vi "CE Examples Navigator.vi"() -> ()   [LabVIEW 2021]
doc: "::: CalcExpress Toolkit :::\nCopyright (c) 2000-2026 Konstantin Shifershteyn. All rights reserved."
uses:
  vi.lib/addons/CalcExpress/cemisc.llb/[ce] CE component paths - Kind of Path Enum.ctl
panel:
  in  "Tree":string(tree) caption="Double-click an example to open"
  in  "Note":string="1)  Interactive Script Processor (CSE ISP) also contains examples. Run it and select Examples menu.\n2)  Many examples use Advanced Analysis VIs. These examples don't work properly if you don't have these VIs."
  out "Description":string
  in  "Mass Compile":bool
  in  "Run CSE ISP":bool
  in  "EXIT":bool
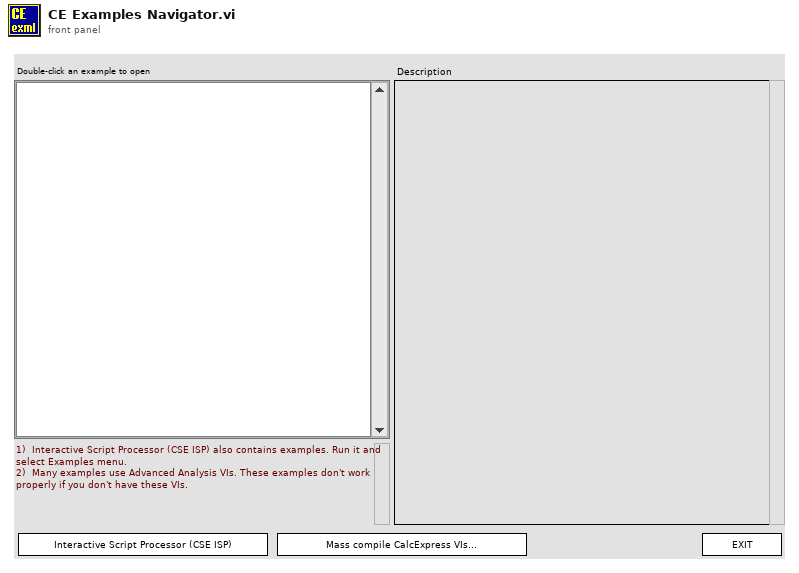
[diagram p1: front panel]
types:
  T1 = typedef "[ce] CE component paths - Kind of Path Enum.ctl" = enum16{"VIs", "FuncVIs", "Help", "Examples", "Project", "Templates"}
  T2 = enum32{"invalid app kind", "Development System", "Run Time System", "Student Edition", "Embedded LabVIEW", "Evaluation", "Custom"}
  T3 = typedef "eventvkey.ctl" = enum16{"ASCII", "Enter", "Return", "Shift", "Ctrl", "Alt", "Cmd", "Opt", "Caps", "NumLock", "Clear", "Break", "Up", "Down", "Left", "Right", "Insert", "Delete", "Home", "End", "PageUp", "PageDown", "Escape", "Help", "Pause", "ScrollLock", "F1", "F2", "F3", "F4", "F5", "F6", "F7", "F8", "F9", "F10", "F11", "F12", "F13", "F14", "F15", "F16", "F17", "F18", "F19", "F20", "F21", "F22", "F23", "F24", "Play", "VolumeUp", "VolumeDown", "Mute", "Two Byte Char"}
  T4 = cluster{"Shift":bool, "Ctrl":bool, "Alt":bool, "Cmd":bool, "Opt":bool}
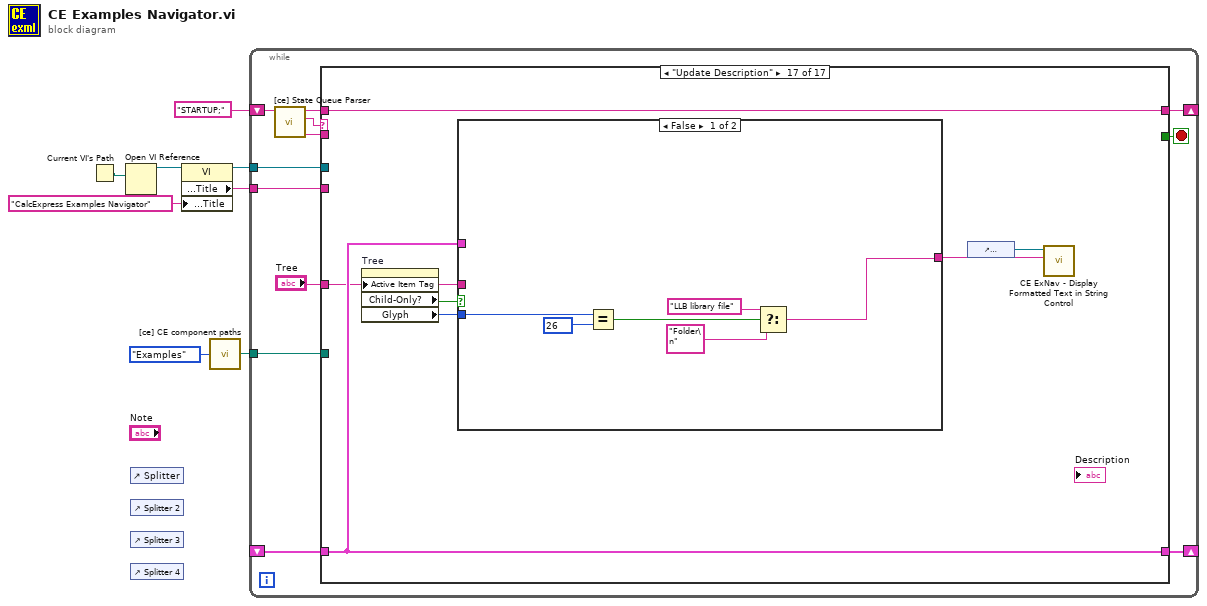
[diagram p0: block diagram]
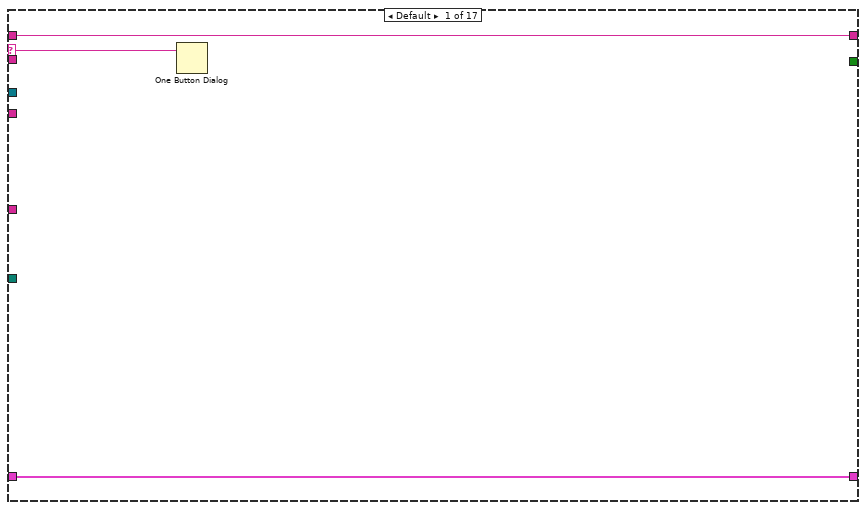
[diagram p2: hidden frame]
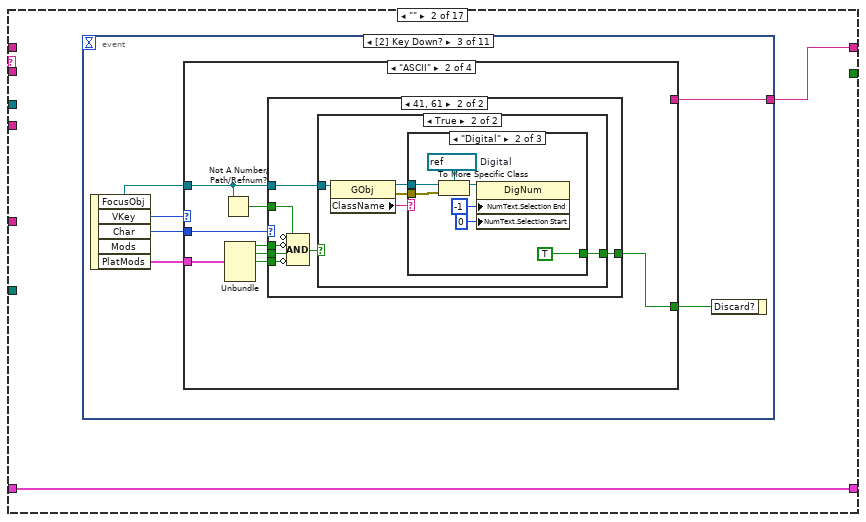
[diagram p3: hidden frame]
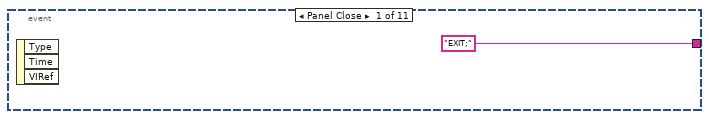
[diagram p4: hidden frame]
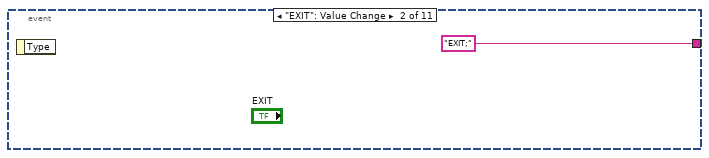
[diagram p5: hidden frame]
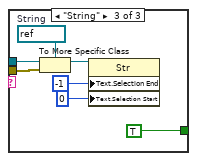
[diagram p10: hidden frame]
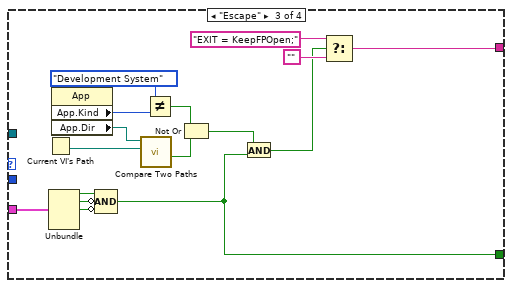
[diagram p11: hidden frame]
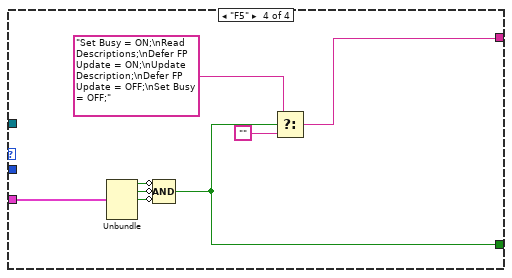
[diagram p12: hidden frame]
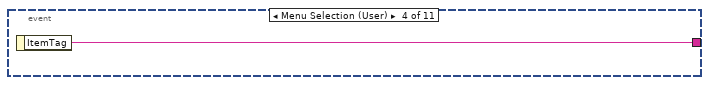
[diagram p13: hidden frame]
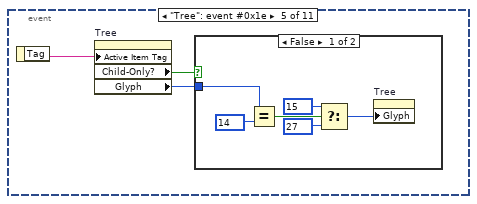
[diagram p14: hidden frame]
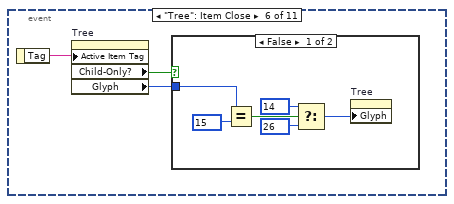
[diagram p16: hidden frame]
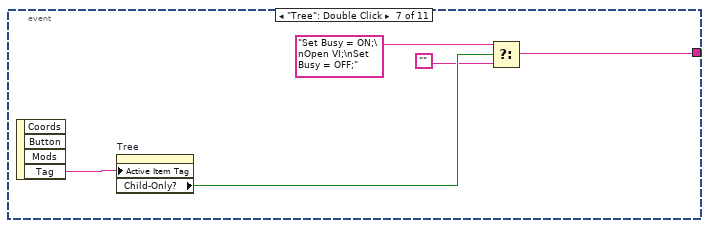
[diagram p18: hidden frame]
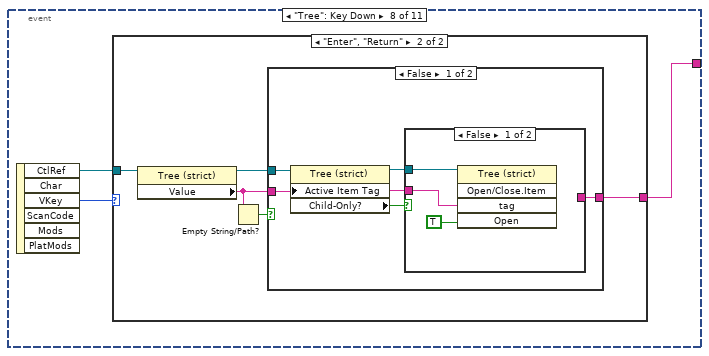
[diagram p19: hidden frame]
diagram:
  n1 = Current VI's Path() -> (path=w6:path)
  n2 = Open VI Reference(vi path=w6) -> (vi reference=w5:refnum<vi>)  [unwired: 5 in, 1 out]
  n3 = control-ref of="Splitter"() -> ()  [unwired: 1 out]
  n4 = control-ref of="Splitter 2"() -> ()  [unwired: 1 out]
  n5 = control-ref of="Splitter 3"() -> ()  [unwired: 1 out]
  n6 = control-ref of="Splitter 4"() -> ()  [unwired: 1 out]
  n7 = property class="VI"(reference=w5, "Front Panel.Title"="CalcExpress Examples Navigator" ("Front Panel Window:Title")) -> (reference out=w4:refnum<vi>, "Front Panel.Title"=w3:string)  [unwired: 1 in, 1 out]
  n8 = call "[ce] CE component paths.vi"("kind of path"=[ce]_CE_component_paths_-_Kind_of_Path_Enum."Examples") -> ("path out"=w7:path)  [unwired: 1 in]
  n9 = while {
    shift-right: [w18] -> _
    shift-left: "STARTUP;" -> [w20]
    tunnel: w7 -> [w14]
    shift-right: [w13] -> _
    shift-left: _ -> [w12]
    tunnel: w4 -> [w10]
    tunnel: w3 -> [w9]
    stop <- w16 stop-if-true
    n10 = call "[ce] State Queue Parser.vi"("input queue"=w20) -> ("state parameters"=w15:string, "state"=w19:string, "remained queue"=w17:string)  [unwired: 6 in]
    n11 = case shown="\"Update Description\"" w19 {
      selector: w19 -> [w22 _ _ _ _ _ _ _ _ _ _ _ _ _ _ _ _]
      tunnel: [w23 w25 "Set Busy = ON;\n\nINIT;\n\nSet Busy = OFF;" w150 w158 w171 w175 w181 w185 w190 w193 w214 w217 w251 w265 w271 w283] -> w18
      tunnel: w17 -> [w23 _ _ w151 w158 w171 w175 w181 w185 w190 w193 w214 w224 w251 w265 w271 w283]
      tunnel: [_ _ _ _ _ TRUE _ _ _ _ _ _ _ _ _ _ _] -> w16
      tunnel: w15 -> [_ _ _ _ _ w169 _ w179 w184 _ w191 _ _ _ _ _ _]
      tunnel: w14 -> [_ _ _ w143 _ _ _ _ _ _ _ _ w223 _ _ _ _]
      tunnel: [w21 w24 w137 w142 w159 w168 w176 w177 w183 w189 w192 w215 w222 w250 w266 w267 w282] -> w13
      tunnel: w12 -> [w21 w24 w137 _ w159 w168 w176 w177 w183 w189 w192 w215 w222 w250 w266 w269 w282]
      tunnel: "Tree" -> [_ _ _ _ _ _ _ _ _ w188 _ _ _ _ _ _ w279]
      tunnel: w10 -> [_ _ _ _ _ w162 _ _ _ _ _ _ _ _ _ _ _]
      tunnel: w9 -> [_ _ _ _ _ w160 _ _ _ _ _ _ _ _ _ _ _]
      frame Default {
        n12 = One Button Dialog(message=w22) -> ()  [unwired: 1 in, 1 out]
      }
      frame "" {
        n13 = event shown="[2] Key Down?" {
          selector: _ -> [_ _ _ _ _ _ _ _ _ _ _]
          dyn-events: _ -> [_ _ _ _ _ _ _ _ _ _ _]
          timeout: _ -> [_ _ _ _ _ _ _ _ _ _ _]
          tunnel: ["EXIT;" "EXIT;" w32 w92 _ _ w113 w116 "Defer FP Update = ON;\nUpdate Description;\nDefer FP Update = OFF;" "Menu = CSE ISP;" ("ItemTag") "Menu = Mass Compile;" ("ItemTag")] -> w25
          event Panel Close {
            n14 = event-data() -> ()  [unwired: 1 in, 3 out]
          }
          event "EXIT": Value Change {
            n15 = event-data() -> ()  [unwired: 1 in, 1 out]
          }
          event Key Down? {
            n16 = event-data() -> ("FocusObj"=w28:refnum<vi>, "VKey"=w30:T3, "Char"=w29:i16, "PlatMods"=w33:T4)  [unwired: 1 in, 1 out]
            n17 = case shown="\"ASCII\"" w30 {
              tunnel: w33 -> [_ w37 w78 w86]
              tunnel: [_ _ w77 w85] -> w32
              tunnel: [_ w35 w69 w84] -> w31
              tunnel: w29 -> [_ w36 _ _]
              tunnel: w28 -> [_ w34 _ _]
              frame Default {
              }
              frame "ASCII" {
                n18 = Not A Number/Path/Refnum?(number/path/refnum=w34) -> (NaN/Path/Refnum?=w41:bool)
                n19 = Unbundle(w37) -> ("Shift"=w38:bool, "Ctrl"=w39:bool, "Alt"=w40:bool)  [unwired: 2 out]
                n20 = case shown="41, 61" w36 {
                  tunnel: w38 -> [_ w48]
                  tunnel: w39 -> [_ w47]
                  tunnel: w40 -> [_ w46]
                  tunnel: w34 -> [_ w44]
                  tunnel: [_ w43] -> w35
                  tunnel: w41 -> [_ w42]
                  frame Default {
                  }
                  frame 65, 97 {
                    n21 = Compound Arithmetic op=AND(invert w42, invert w48, w47, invert w46) -> (w45:bool)
                    n22 = case shown="True" w45 {
                      tunnel: w44 -> [_ w53]
                      tunnel: [_ w51] -> w43
                      frame False {
                      }
                      frame True {
                        n23 = property class="GObj"(reference=w53) -> (reference out=w50:refnum<vi>, error out=w49:errorcluster, "ClassName"=w52:string)  [unwired: 1 in]
                        n24 = case shown="\"Digital\"" w52 {
                          tunnel: [_ TRUE TRUE] -> w51
                          tunnel: w50 -> [_ w58 w65]
                          tunnel: w49 -> [_ w57 w64]
                          frame Default {
                          }
                          frame "Digital" {
                            w59 = refnum<vi> refnum  # Digital
                            n25 = To More Specific Class(target class=w59, reference=w58, error in=w57) -> (specific class reference=w56:refnum<vi>)  [unwired: 1 out]
                            n26 = property class="DigNum"(reference=w56, "NumText.Selection End"=-1 ("Numeric Text.Selection:End"), "NumText.Selection Start"=u32 0 ("Numeric Text.Selection:Start")) -> ()  [unwired: 1 in, 2 out]
                          }
                          frame "String" {
                            w66 = refnum<vi> refnum  # String
                            n27 = To More Specific Class(target class=w66, reference=w65, error in=w64) -> (specific class reference=w63:refnum<vi>)  [unwired: 1 out]
                            n28 = property class="Str"(reference=w63, "Text.Selection End"=-1 ("Numeric Text.Selection:End"), "Text.Selection Start"=u32 0 ("Numeric Text.Selection:Start")) -> ()  [unwired: 1 in, 2 out]
                          }
                        }
                      }
                    }
                  }
                }
              }
              frame "Escape" {
                n29 = Current VI's Path() -> (path=w76:path)
                n30 = Unbundle(w78) -> ("Shift"=w79:bool, "Ctrl"=w80:bool, "Alt"=w81:bool)  [unwired: 2 out]
                n31 = property class="App"() -> ("App.Kind"=w74:T2, "App.Dir"=w75:path)  [unwired: 2 in, 2 out]
                n32 = Compound Arithmetic op=AND(w79, invert w80, invert w81) -> (w69:bool)
                n33 = call <vilib>:"Compare Two Paths.vi"("Path 2"=w76, "Path 1"=w75) -> ("Path 2 Relative to Path 1?"=w72:bool)  [unwired: 6 in, 3 out]
                n34 = Not Equal?(x=T2."Development System", y=w74) -> (x != y?=w73:bool)
                n35 = Not Or(1:w72, 2:w73) -> (0:w71:bool)
                n36 = And(x=w71, y=w69) -> (x .and. y?=w68:bool)
                n37 = Select(t="EXIT = KeepFPOpen;", s=w68, f="") -> (s? t:f=w77:string)
              }
              frame "F5" {
                n38 = Unbundle(w86) -> ("Shift"=w87:bool, "Ctrl"=w88:bool, "Alt"=w89:bool)  [unwired: 2 out]
                n39 = Compound Arithmetic op=AND(invert w87, invert w88, invert w89) -> (w84:bool)
                n40 = Select(t="Set Busy = ON;\nRead Descriptions;\nDefer FP Update = ON;\nUpdate Description;\nDefer FP Update = OFF;\nSet Busy = OFF;", s=w84, f="") -> (s? t:f=w85:string)
              }
            }
            n41 = event-data("Discard?"=w31) -> ()  [unwired: 1 in, 1 out]
          }
          event Menu Selection (User) {
            n42 = event-data() -> ("ItemTag"=w92:string)  [unwired: 1 in]
          }
          event "Tree": event #0x1e {
            n43 = event-data() -> ("Tag"=w95:string)  [unwired: 1 in]
            n44 = property on="Tree" class="Tree (strict)"("Active Item Tag"=w95) -> ("Child-Only?"=w93:bool, "Glyph"=w94:i32)  [unwired: 2 in, 2 out]
            n45 = case shown="False" w93 {
              tunnel: w94 -> [w101 _]
              frame False {
                n46 = Equal?(x=w101, y=14) -> (x = y?=w99:bool)
                n47 = Select(t=15, s=w99, f=27) -> (s? t:f=w98:i32)
                n48 = property on="Tree" class="Tree (strict)"("Glyph"=w98) -> ()  [unwired: 2 in, 2 out]
              }
              frame True {
              }
            }
          }
          event "Tree": Item Close {
            n49 = event-data() -> ("Tag"=w102:string)  [unwired: 1 in]
            n50 = property on="Tree" class="Tree (strict)"("Active Item Tag"=w102) -> ("Child-Only?"=w103:bool, "Glyph"=w104:i32)  [unwired: 2 in, 2 out]
            n51 = case shown="False" w103 {
              tunnel: w104 -> [w110 _]
              frame False {
                n52 = Equal?(x=w110, y=15) -> (x = y?=w108:bool)
                n53 = Select(t=14, s=w108, f=26) -> (s? t:f=w107:i32)
                n54 = property on="Tree" class="Tree (strict)"("Glyph"=w107) -> ()  [unwired: 2 in, 2 out]
              }
              frame True {
              }
            }
          }
          event "Tree": Double Click {
            n55 = event-data() -> ("Tag"=w115:string)  [unwired: 1 in, 3 out]
            n56 = property on="Tree" class="Tree (strict)"("Active Item Tag"=w115) -> ("Child-Only?"=w114:bool)  [unwired: 2 in, 2 out]
            n57 = Select(t="Set Busy = ON;\nOpen VI;\nSet Busy = OFF;", s=w114, f="") -> (s? t:f=w113:string)
          }
          event "Tree": Key Down {
            n58 = event-data() -> ("CtlRef"=w118:refnum<vi>, "VKey"=w117:T3)  [unwired: 1 in, 4 out]
            n59 = case shown="\"Enter\", \"Return\"" w117 {
              tunnel: w118 -> [_ w123]
              tunnel: [_ w119] -> w116
              frame Default {
              }
              frame "Enter", "Return" {
                n60 = property class="Tree (strict)"(reference=w123) -> (reference out=w122:refnum<vi>, "Value"=w120:string)  [unwired: 1 in, 1 out]
                n61 = Empty String/Path?(string/path=w120) -> (empty?=w121:bool)
                n62 = case shown="False" w121 {
                  tunnel: w122 -> [w128 _]
                  tunnel: w120 -> [w124 _]
                  tunnel: [w125 _] -> w119
                  frame False {
                    n63 = property on="Property Node" class="Tree (strict)"(reference=w128, "Active Item Tag"=w124) -> (reference out=w127:refnum<vi>, "Child-Only?"=w126:bool)  [unwired: 1 in, 1 out]
                    n64 = case shown="False" w126 {
                      tunnel: w127 -> [w131 _]
                      tunnel: [_ "Set Busy = ON;\nOpen VI;\nSet Busy = OFF;"] -> w125
                      tunnel: w124 -> [w129 _]
                      frame False {
                        n65 = invoke class="Tree (strict)" method="Open/Close.Item"(reference=w131, "tag"=w129, "Open"=TRUE) -> ()  [unwired: 2 in, 5 out]
                      }
                      frame True {
                      }
                    }
                  }
                  frame True {
                  }
                }
              }
            }
          }
          event "Tree": Value Change {
            (unwired) "Set Busy = ON;\nUpdate Description;\nSet Busy = OFF;"
            n66 = event-data() -> ()  [unwired: 1 in, 2 out]
          }
          event "Run CSE ISP": Value Change {
            n67 = event-data() -> ()  [unwired: 1 in, 1 out]
          }
          event "Mass Compile": Value Change {
            n68 = event-data() -> ()  [unwired: 1 in, 1 out]
          }
        }
      }
      frame "STARTUP" {
      }
      frame "INIT" {
        n69 = Build Array("[ex ce*.vi" ("pattern"), "FuncVI-*.vi" ("pattern")) -> (w146:string[])
        n70 = for {
          tunnel: w143 -> [w157]
          tunnel: w146 -> [w155] mode=indexing
          shift-right: [w152] -> w148
          shift-left: path[] [] -> [w153]
          n71 = call <vilib>:"Recursive File List.vi"("pattern"=w155, "Treat LLBs as Folders?"=TRUE, "Folder Path"=w157) -> ("All Files in Dir"=w154:path[])  [unwired: 4 in, 4 out]
          n72 = Build Array (concatenate)(w153, w154) -> (w152:path[])
        }
        n73 = Sort 1D Array(array=w148) -> (sorted array=w139:path[])
        n74 = Array Size(array=w139) -> (size(s)=w140:i32)
        n75 = Initialize Array("", w140) -> (w138:string[])
        n76 = Bundle(w139, w138) -> (w142:cluster{path[], string[]})  [unwired: 1 in]
        n77 = Concatenate Strings("Defer FP Update = ON;\nRead Descriptions;\nBuild Tree;\nDefer FP Update = OFF;\n\nInit Done;", w151) -> (w150:string)
      }
      frame "INIT Done" {
      }
      frame "EXIT" {
        n78 = property class="VI"(reference=w162, "Front Panel.Title"=w160) -> (reference out=w161:refnum<vi>)  [unwired: 1 in, 1 out]
        n79 = case shown="Default" w169 {
          tunnel: w161 -> [w172 w174]
          tunnel: [w172 w173] -> w164
          frame "KeepFPOpen" {
          }
          frame Default {
            n80 = invoke class="VI" method="FP.Close"(reference=w174) -> (reference out=w173:refnum<vi>)  [unwired: 2 in, 2 out]
          }
        }
        n81 = local write "Description"("") -> ()
        n82 = invoke on="Tree" class="Tree (strict)" method="Edit Tree Items.Delete"("tag"="", "Delete Children"=TRUE ("Delete Children?")) -> (error out=w163:errorcluster)  [unwired: 3 in, 4 out]
        n83 = Close Reference(reference=w164, error in (no error)=w163) -> ()  [unwired: 1 out]
      }
      frame "---------------------------------- 1" {
      }
      frame "Defer FP Update" {
        n84 = case shown="\"ON\"" w179 {
          tunnel: [_ TRUE] -> w178
          frame "OFF", Default {
          }
          frame "ON" {
          }
        }
        n85 = property class="VI"() -> ("Front Panel"=w180:refnum<vi>)  [unwired: 2 in, 2 out]
        n86 = property class="Pnl"(reference=w180, "Defer Panel Updates"=w178) -> ()  [unwired: 1 in, 2 out]
      }
      frame "Set Busy" {
        n87 = case shown="\"ON\"" w184 {
          frame "OFF", Default {
            n88 = call <vilib>:"Unset Busy.vi"() -> ()  [unwired: 11 in, 1 out]
          }
          frame "ON" {
            n89 = call <vilib>:"Set Busy.vi"() -> ()  [unwired: 10 in, 2 out]
          }
        }
      }
      frame "Open VI" {
        n90 = String To Path(string=w188) -> (path=w186:path)
        n91 = call "CE ExNav - VIs Control.vi"("cmd"=enum16{"open", "run", "description"}."open", "VI path"=w186) -> ()  [unwired: 8 in, 2 out]
      }
      frame "Menu" {
        n92 = case shown="\"About\"" w191 {
          frame Default {
          }
          frame "About" {
            n93 = call "[ce] MsgBox - About CalcExpress.vi"() -> ()  [unwired: 11 in, 1 out]
          }
          frame "CE Help" {
            n94 = call "[ce] CE component paths.vi"("kind of path"=[ce]_CE_component_paths_-_Kind_of_Path_Enum."Help", "append path"="CEToolkit.chm" ("append")) -> ("path out"=w196:path)
            n95 = Control Online Help(2:w196, 4:enum16{"Contents", "Key", "Close"}."Contents" ("Operation")) -> (0:w197:errorcluster)  [unwired: 2 in]
            n96 = call <vilib>:"Simple Error Handler.vi"("error in (no error)"=w197) -> ()  [unwired: 4 in, 5 out]
          }
          frame "CSE ISP" {
            n97 = call "[ce] CE component paths.vi"("kind of path"=[ce]_CE_component_paths_-_Kind_of_Path_Enum."Project", "append path"="CSE ISP.vi" ("append")) -> ("path out"=w200:path)
            n98 = call "CE ExNav - VIs Control.vi"("cmd"=enum16{"open", "run", "description"}."run", "VI path"=w200) -> ("error out"=w202:errorcluster)  [unwired: 8 in, 1 out]
            n99 = call <vilib>:"Simple Error Handler.vi"("error in (no error)"=w202) -> ()  [unwired: 4 in, 5 out]
          }
          frame "VarMan Spy" {
            n100 = call "[ce] CE component paths.vi"("kind of path"=[ce]_CE_component_paths_-_Kind_of_Path_Enum."Project", "append path"="VarMan Spy.vi" ("append")) -> ("path out"=w208:path)
            n101 = call "CE ExNav - VIs Control.vi"("cmd"=enum16{"open", "run", "description"}."run", "VI path"=w208) -> ("error out"=w206:errorcluster)  [unwired: 8 in, 1 out]
            n102 = call <vilib>:"Simple Error Handler.vi"("error in (no error)"=w206) -> ()  [unwired: 4 in, 5 out]
          }
          frame "Mass Compile" {
            n103 = call "[ce] CE component paths.vi"("kind of path"=[ce]_CE_component_paths_-_Kind_of_Path_Enum."Project", "append path"="Mass Compile CalcExpress VIs.vi" ("append")) -> ("path out"=w213:path)
            n104 = call "CE ExNav - VIs Control.vi"("cmd"=enum16{"open", "run", "description"}."run", "VI path"=w213) -> ("error out"=w211:errorcluster)  [unwired: 8 in, 1 out]
            n105 = call <vilib>:"Simple Error Handler.vi"("error in (no error)"=w211) -> ()  [unwired: 4 in, 5 out]
          }
        }
      }
      frame "---------------------------------- 2" {
      }
      frame "Build Tree" {
        n106 = Unbundle(w222) -> (w221:path[])  [unwired: 1 out]
        n107 = invoke on="Tree" class="Tree (strict)" method="Edit Tree Items.Delete"("tag"="", "Delete Children"=TRUE ("Delete Children?")) -> (error out=w218:errorcluster)  [unwired: 3 in, 4 out]
        n108 = for {
          tunnel: w221 -> [w229] mode=indexing
          tunnel: w223 -> [w226]
          tunnel: w218 -> [_]
          n109 = Path To String(path=w226) -> (string=w225:string)
          n110 = call <vilib>:"Compare Two Paths.vi"("Path 2"=w229, "Path 1"=w226) -> ("Relative Path from 1 to 2"=w228:path)  [unwired: 6 in, 3 out]
          n111 = Path to Array of Strings(0:w228) -> (2:w227:string[])  [unwired: 1 out]
          n112 = for {
            N -> [w232]
            tunnel: w227 -> [w240] mode=indexing
            shift-right: [w241] -> _
            shift-left: w225 -> [w237]
            i -> [w233]
            n113 = Decrement(x=w232) -> (x-1=w231:i32)
            n114 = Concatenate Strings(w237, "\\" ("string"), w240) -> (w235:string)
            n115 = Equal?(x=w231, y=w233) -> (x = y?=w230:bool)
            n116 = Equal To 0?(x=w233) -> (x = 0?=w238:bool)
            n117 = property on="Tree" class="Tree (strict)"("Active Item Tag"=w235) -> (error out=w234:errorcluster)  [unwired: 2 in, 1 out]
            n118 = Select(t="", s=w238, f=w237) -> (s? t:f=w239:string)
            n119 = case shown="No Error" w234 {
              tunnel: [w243 w249] -> w241
              tunnel: w240 -> [_ w248]
              tunnel: w239 -> [_ w246]
              tunnel: w235 -> [w243 w245]
              tunnel: w230 -> [_ w244]
              frame No Error {
              }
              frame Error {
                n120 = invoke on="Tree" class="Tree (strict)" method="Edit Tree Items.Add Item"("Parent Tag"=w246, "Child Position"=-1, "Left Cell"=w248, "Child Tag"=w245, "Child Only?"=w244) -> ("Edit Tree Items:Add Item"=w249:string)  [unwired: 4 in, 8 out]
              }
            }
          }
        }
        n121 = Concatenate Strings("Build Tree 2;" ("string"), w224) -> (w217:string)
      }
      frame "Build Tree 2" {
        n122 = invoke on="Tree" class="Tree (strict)" method="Open/Close.Open/Close All"("Open"=FALSE ("Open?")) -> (error out=w252:errorcluster)  [unwired: 3 in, 3 out]
        n123 = property on="Tree" class="Tree (strict)"(error in=w252) -> ("All Tags"=w254:string[])  [unwired: 1 in, 2 out]
        n124 = for {
          tunnel: w254 -> [w259] mode=indexing
          n125 = String To Path(string=w259) -> (path=w260:path)
          n126 = property on="Tree" class="Tree (strict)"("Active Item Tag"=w259) -> (error out=w262:errorcluster, "Child-Only?"=w264:bool)  [unwired: 2 in, 1 out]
          n127 = File/Directory Info(path=w260) -> (directory=w258:bool)  [unwired: 1 in, 6 out]
          n128 = Select(t=14, s=w258, f=26) -> (s? t:f=w257:i32)
          n129 = Select(t=21, s=w264, f=w257) -> (s? t:f=w261:i32)
          n130 = property on="Tree" class="Tree (strict)"(error in=w262, "Glyph"=w261) -> ()  [unwired: 1 in, 2 out]
        }
      }
      frame "---------------------------------- 3" {
      }
      frame "Read Descriptions" {
        n131 = Unbundle(w269) -> (w270:path[])  [unwired: 1 out]
        n132 = for {
          tunnel: w270 -> [w275] mode=indexing
          tunnel: [w273] -> w268 mode=indexing
          n133 = call "CE ExNav - VIs Control.vi"("cmd"=enum16{"open", "run", "description"}."description", "VI path"=w275) -> ("description"=w274:string)  [unwired: 8 in, 1 out]
          n134 = Match Pattern(string=w274, regular expression="\\n:::") -> (before substring=w273:string)  [unwired: 1 in, 3 out]
        }
        n135 = Bundle(cluster=w269, w268) -> (w267:cluster{path[], string[]})  [unwired: 1 in]
      }
      frame "Update Description" {
        n136 = property on="Tree" class="Tree (strict)"("Active Item Tag"=w279) -> ("Child-Only?"=w278:bool, "Glyph"=w277:i32)  [unwired: 2 in, 2 out]
        n137 = case shown="False" w278 {
          tunnel: w282 -> [_ w306]
          tunnel: [w287 w291] -> w280
          tunnel: w279 -> [_ w290]
          tunnel: w277 -> [w286 _]
          frame False {
            n138 = Equal?(x=w286, y=26) -> (x = y?=w284:bool)
            n139 = Select(t="LLB library file", s=w284, f="Folder\n") -> (s? t:f=w287:string)
          }
          frame True {
            n140 = Unbundle(w306) -> (w305:path[], w303:string[])
            n141 = String To Path(string=w290) -> (path=w296:path)
            n142 = Search 1D Array(1D array=w305, element=w296) -> (index of element=w304:i32)  [unwired: 1 in]
            n143 = Index Array(array=w303, index=w304) -> (element=w297:string)
            n144 = Strip Path(path=w296) -> (name=w295:string)  [unwired: 1 out]
            n145 = Empty String/Path?(string/path=w297) -> (empty?=w302:bool)
            n146 = Not(x=w302) -> (.not. x?=w301:bool)
            n147 = Format Into String(format string="<B>%s</B>\n\n", w295) -> (resulting string=w293:string)  [unwired: 2 in, 1 out]
            n148 = Match Pattern(string=w297, regular expression="^<[Bb]>") -> (offset past match=w298:i32)  [unwired: 1 in, 3 out]
            n149 = Select(t=w297, s=w301, f="This is example of using CalcExpress VIs.\n") -> (s? t:f=w292:string)
            n150 = case shown="..-1" w298 {
              tunnel: w293 -> [w309 _]
              tunnel: w292 -> [w308 w310]
              tunnel: [w307 w310] -> w291
              frame ..-1 {
                n151 = Concatenate Strings(w309, w308) -> (w307:string)
              }
              frame 0.. {
              }
            }
          }
        }
        n152 = control-ref of="Description"() -> (w281:refnum<vi>)
        n153 = call "CE ExNav - Display Formatted Text in String Control.vi"("Formatted text"=w280, "Str Refnum"=w281) -> ()  [unwired: 8 in, 2 out]
      }
    }
  }
